vi "ATM Grafted.vi"() -> ()   [LabVIEW 2026]
doc: "ATM controller (CLD 100928D-01). Starts the Account Manager DQMH module, sets the start state through Initialize ATM Session.vi (session controls disabled, Welcome message) and runs a producer/consumer pair. The producer loop handles the panel events (Card Simulator, Enter, Left Buttons, Right Buttons, typing in User Input) and sends each as a command WITH its data (the User Input text, the pressed button index) over a queue. The consumer loop passes every command to Handle ATM Command.vi and writes ATM Messages, Left Menu and Right Menu. While a card is inserted the consumer waits at most 10 s for a command; a timeout terminates the session. When the controller asks to stop, the Card Simulator is released, the producer ends, the queue is released and the module is stopped. Accounts.txt is read from the folder of this VI. All errors are merged into error out."
uses:
  Libraries/Account Manager/Account Manager.lvlib
panel:
  out "error out":errorcluster
  in  "Enter":bool
  in  "User Input":string
  in  "Right Buttons":T1
  out "Right Menu":T2
  in  "Left Buttons":T1
  out "Left Menu":T2
  in  "Card Simulator":bool
  out "ATM Messages":string
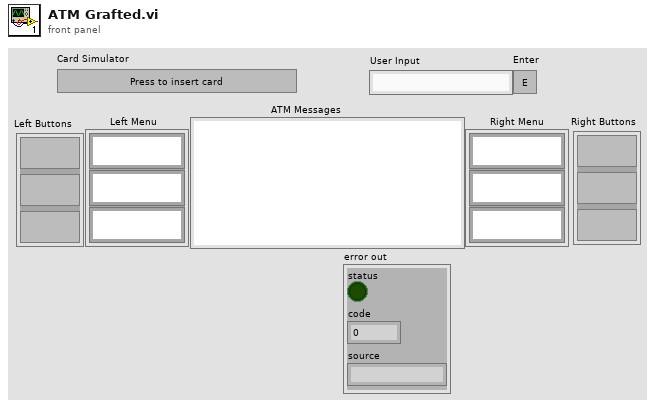
[diagram p1: front panel]
types:
  T1 = cluster{"Func Button":bool, "Func Button 2":bool, "Func Button 3":bool}
  T2 = cluster{"RFS String":string, "RFS String 2":string, "RFS String 3":string}
  T3 = cluster{"Accounts File":path, "Card Inserted":bool, "Account Number":string, "First Name":string, "Last Name":string, "Menu":string, "Pending":string, "Message":string}
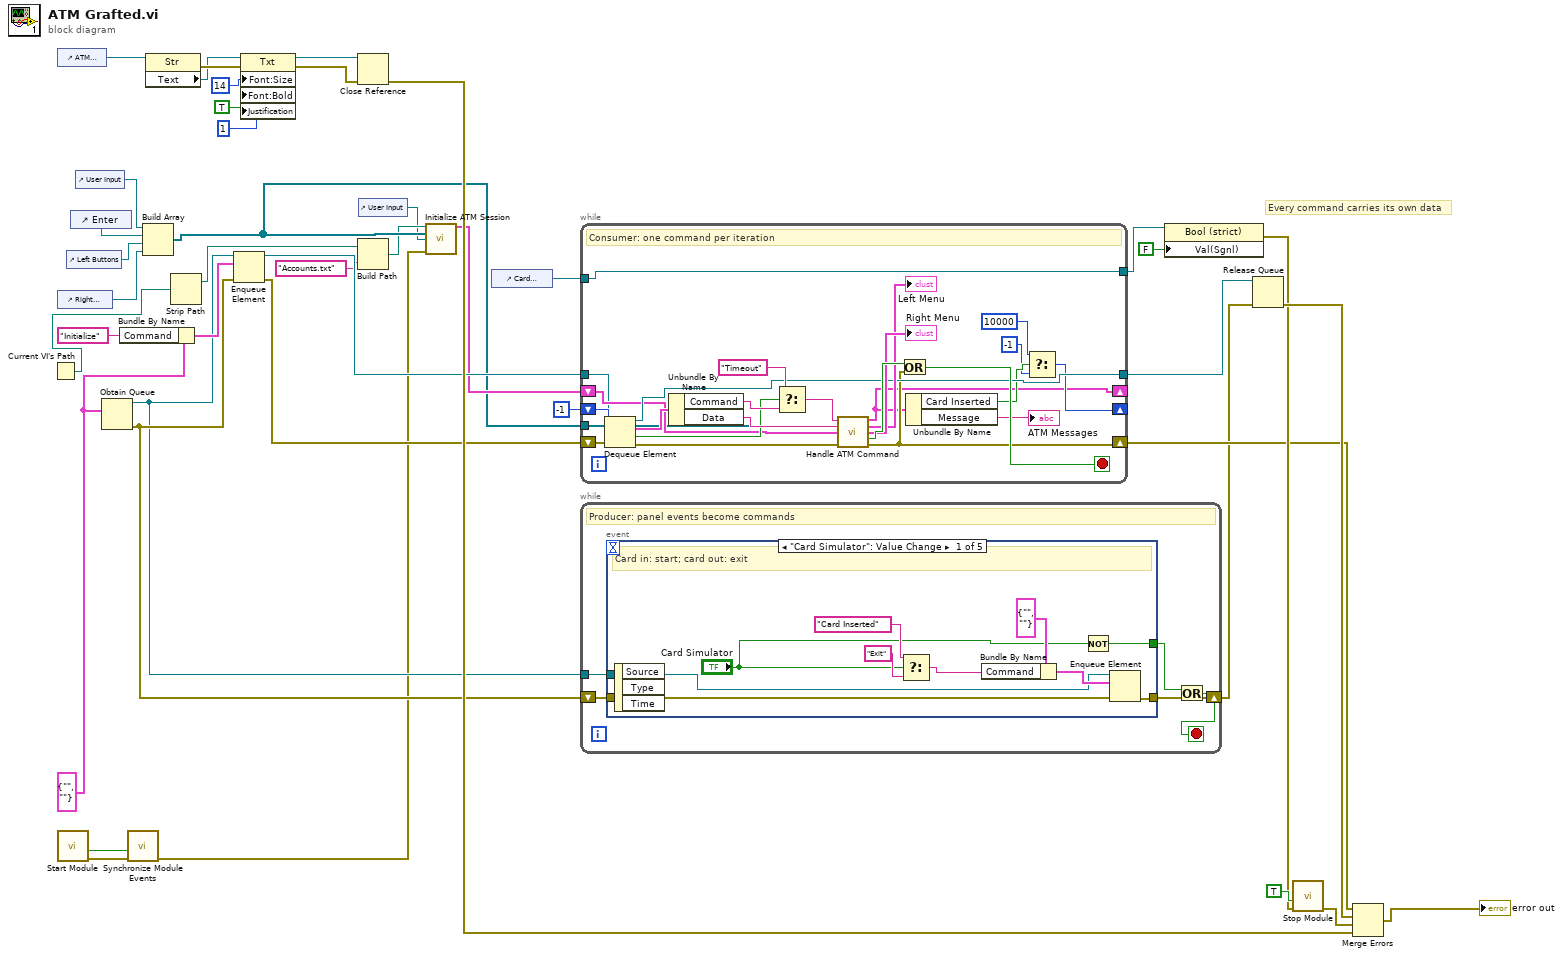
[diagram p0: block diagram]
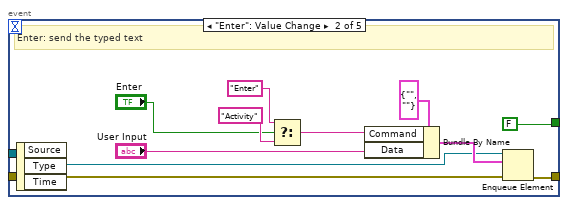
[diagram p2: hidden frame]
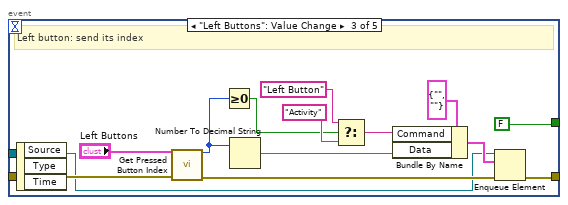
[diagram p3: hidden frame]
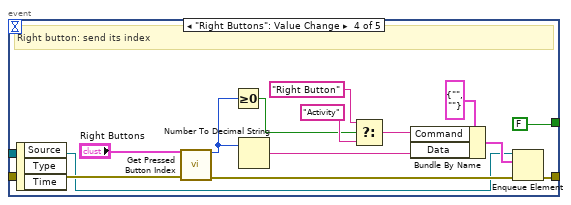
[diagram p4: hidden frame]
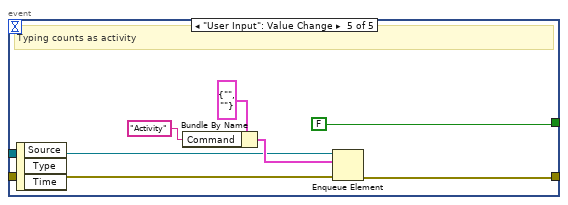
[diagram p5: hidden frame]
diagram:
  w17 = cluster{"Command":string, "Data":string} {"Command"="", "Data"=""} ("Command Type")
  # "Every command carries its own data"
  n1 = Current VI's Path() -> (path=w11:path)
  n2 = control-ref of="ATM Messages"() -> (w1:refnum<vi>)
  n3 = control-ref of="Right Buttons"() -> (w6:refnum<vi>)
  n4 = call "Start Module.vi"() -> ("error out"=w8:errorcluster, "Wait for Event Sync?"=w9:bool)  [unwired: 7 in, 3 out]
  n5 = control-ref of="Left Buttons"() -> (w5:refnum<vi>)
  n6 = control-ref of="Enter"() -> (w4:refnum<vi>)
  n7 = control-ref of="User Input"() -> (w3:refnum<vi>)
  n8 = Obtain Queue(element data type=w17) -> (queue out=w18:refnum<queue>, error out=w19:errorcluster)  [unwired: 4 in, 1 out]
  n9 = Bundle By Name(cluster=w17, "Command"="Initialize" ("Initialize Command")) -> (w21:cluster{"Command":string, "Data":string})
  n10 = call "Synchronize Module Events.vi"("error in"=w8, "Wait for Event Sync?"=w9) -> ("error out"=w10:errorcluster)  [unwired: 9 in]
  n11 = Build Array(w3, w4, w5, w6) -> (w15:refnum<vi>[])
  n12 = property class="Str"(reference=w1) -> (error out=w25:errorcluster, "Text"=w24:refnum<vi>)  [unwired: 1 in, 1 out]
  n13 = Strip Path(path=w11) -> (stripped path=w12:path)  [unwired: 1 out]
  n14 = Enqueue Element(queue=w18, element=w21, error in (no error)=w19) -> (queue out=w22:refnum<queue>, error out=w23:errorcluster)  [unwired: 1 in, 1 out]
  n15 = property class="Txt"(reference=w24, error in=w25, "Font:Size"=14 ("Font Size"), "Font:Bold"=TRUE ("Bold"), "Justification"=1 ("Centred")) -> (reference out=w29:refnum<vi>, error out=w30:errorcluster)
  n16 = Close Reference(reference=w29, error in (no error)=w30) -> (error out=w31:errorcluster)
  n17 = Build Path(base path=w12, name or relative path="Accounts.txt" ("Accounts File Name")) -> (appended path=w14:path)
  n18 = control-ref of="User Input"() -> (w2:refnum<vi>)
  n19 = call "Initialize ATM Session.vi"("Accounts File"=w14, "Controls"=w15, "User Input Ref"=w2, "error in"=w10) -> ("Session out"=w16:T3)  [unwired: 10 in, 1 out]
  n20 = control-ref of="Card Simulator"() -> (w7:refnum<vi>)
  n21 = while {
    tunnel: w7 -> [w45]
    shift-right: [w49] -> _
    shift-left: -1 ("No Card Wait Forever") -> [w48]
    tunnel: w15 -> [w44]
    tunnel: [w45] -> w36
    tunnel: w22 -> [w43]
    shift-right: [w51] -> w34
    shift-left: w23 -> [w50]
    shift-right: [w47] -> _
    shift-left: w16 -> [w46]
    tunnel: [w55] -> w35
    stop <- w67 stop-if-true
    # "Consumer: one command per iteration"
    n22 = Dequeue Element(queue=w43, timeout in ms (-1)=w48, error in (no error)=w50) -> (queue out=w55:refnum<queue>, element=w56:cluster{"Command":string, "Data":string}, timed out?=w57:bool, error out=w58:errorcluster)
    n23 = Unbundle By Name(w56) -> ("Command"=w59:string, "Data"=w60:string)
    n24 = Select(t="Timeout" ("Timeout Command"), s=w57, f=w59) -> (s? t:f=w62:string)
    n25 = call "Handle ATM Command.vi"("Command"=w62, "Data"=w60, "Session in"=w46, "Controls"=w44, "error in"=w58) -> ("Session out"=w47:T3, "Left Menu"=→"Left Menu":T2, "Right Menu"=→"Right Menu":T2, "Stop"=w65:bool, "error out"=w51:errorcluster)  [unwired: 6 in]
    n26 = Or(x=w65, y=w51) -> (x .or. y?=w67:bool)
    n27 = Unbundle By Name(w47) -> ("Card Inserted"=w54:bool, "Message"=→"ATM Messages":string)
    n28 = Select(t=10000 ("Inactivity Timeout ms"), s=w54, f=-1 ("Wait Forever")) -> (s? t:f=w49:i32)
  }
  n29 = while {
    tunnel: w18 -> [w68]
    shift-right: [w70] -> w32
    shift-left: w19 -> [w69]
    stop <- w72 stop-if-true
    # "Producer: panel events become commands"
    n30 = event shown="[0] \"Card Simulator\": Value Change" {
      selector: _ -> [_ _ _ _ _]
      dyn-events: _ -> [_ _ _ _ _]
      timeout: _ -> [_ _ _ _ _]
      tunnel: [w82 FALSE ("Enter Go On") FALSE ("Left Go On") FALSE ("Right Go On") FALSE ("Typing Go On")] -> w71
      tunnel: w68 -> [w73 w83 w94 w108 w122]
      tunnel: w69 -> [w74 w84 w95 w109 w123]
      tunnel: [w81 w92 w106 w120 w127] -> w70
      event "Card Simulator": Value Change {
        # "Card in: start; card out: exit"
        n31 = event-data() -> ()  [unwired: 1 in, 3 out]
        n32 = Select(t="Card Inserted" ("Card Inserted Command"), s="Card Simulator", f="Exit" ("Exit Command")) -> (s? t:f=w78:string)
        n33 = Bundle By Name(cluster=cluster{"Command":string, "Data":string} {"Command"="", "Data"=""} ("Card Command Type"), "Command"=w78) -> (w80:cluster{"Command":string, "Data":string})
        n34 = Not(x="Card Simulator") -> (.not. x?=w82:bool)
        n35 = Enqueue Element(queue=w73, element=w80, error in (no error)=w74) -> (error out=w81:errorcluster)  [unwired: 1 in, 2 out]
      }
      event "Enter": Value Change {
        # "Enter: send the typed text"
        n36 = event-data() -> ()  [unwired: 1 in, 3 out]
        n37 = Select(t="Enter" ("Enter Command"), s="Enter", f="Activity" ("Enter Activity Command")) -> (s? t:f=w89:string)
        n38 = Bundle By Name(cluster=cluster{"Command":string, "Data":string} {"Command"="", "Data"=""} ("Enter Command Type"), "Command"=w89, "Data"="User Input") -> (w91:cluster{"Command":string, "Data":string})
        n39 = Enqueue Element(queue=w83, element=w91, error in (no error)=w84) -> (error out=w92:errorcluster)  [unwired: 1 in, 2 out]
      }
      event "Left Buttons": Value Change {
        # "Left button: send its index"
        n40 = event-data() -> ()  [unwired: 1 in, 3 out]
        n41 = call "Get Pressed Button Index.vi"("Buttons"="Left Buttons", "error in"=w95) -> ("Index"=w97:i32, "error out"=w98:errorcluster)  [unwired: 12 in]
        n42 = Greater Or Equal To 0?(x=w97) -> (x >= 0?=w99:bool)
        n43 = Number To Decimal String(number=w97) -> (decimal integer string=w103:string)  [unwired: 1 in]
        n44 = Select(t="Left Button" ("Left Button Command"), s=w99, f="Activity" ("Left Activity Command")) -> (s? t:f=w102:string)
        n45 = Bundle By Name(cluster=cluster{"Command":string, "Data":string} {"Command"="", "Data"=""} ("Left Command Type"), "Command"=w102, "Data"=w103) -> (w105:cluster{"Command":string, "Data":string})
        n46 = Enqueue Element(queue=w94, element=w105, error in (no error)=w98) -> (error out=w106:errorcluster)  [unwired: 1 in, 2 out]
      }
      event "Right Buttons": Value Change {
        # "Right button: send its index"
        n47 = event-data() -> ()  [unwired: 1 in, 3 out]
        n48 = call "Get Pressed Button Index.vi"("Buttons"="Right Buttons", "error in"=w109) -> ("Index"=w111:i32, "error out"=w112:errorcluster)  [unwired: 12 in]
        n49 = Greater Or Equal To 0?(x=w111) -> (x >= 0?=w113:bool)
        n50 = Number To Decimal String(number=w111) -> (decimal integer string=w117:string)  [unwired: 1 in]
        n51 = Select(t="Right Button" ("Right Button Command"), s=w113, f="Activity" ("Right Activity Command")) -> (s? t:f=w116:string)
        n52 = Bundle By Name(cluster=cluster{"Command":string, "Data":string} {"Command"="", "Data"=""} ("Right Command Type"), "Command"=w116, "Data"=w117) -> (w119:cluster{"Command":string, "Data":string})
        n53 = Enqueue Element(queue=w108, element=w119, error in (no error)=w112) -> (error out=w120:errorcluster)  [unwired: 1 in, 2 out]
      }
      event "User Input": Value Change {
        # "Typing counts as activity"
        n54 = event-data() -> ()  [unwired: 1 in, 3 out]
        n55 = Bundle By Name(cluster=cluster{"Command":string, "Data":string} {"Command"="", "Data"=""} ("Typing Command Type"), "Command"="Activity" ("Typing Activity Command")) -> (w126:cluster{"Command":string, "Data":string})
        n56 = Enqueue Element(queue=w122, element=w126, error in (no error)=w123) -> (error out=w127:errorcluster)  [unwired: 1 in, 2 out]
      }
    }
    n57 = Or(x=w71, y=w70) -> (x .or. y?=w72:bool)
  }
  n58 = property class="Bool (strict)"(reference=w36, "Val(Sgnl)"=FALSE ("Card Released")) -> (error out=w38:errorcluster)  [unwired: 1 in, 1 out]
  n59 = Release Queue(queue=w35, error in (no error)=w32) -> (error out=w39:errorcluster)  [unwired: 1 in, 2 out]
  n60 = call "Stop Module.vi"("error in"=w38, "Wait for Module to Stop? (F)"=TRUE ("Wait for Module to Stop")) -> ("error out"=w41:errorcluster)  [unwired: 9 in]
  n61 = Merge Errors(w34, w39, w41, w31) -> (→"error out":errorcluster)
